vi "Condition.vi"(8 "error in":errorcluster, 11 "Actor in":refnum<class "Actor.lvclass">) -> (0 "error out":errorcluster, 3 "Actor out":refnum<class "Actor.lvclass">)   [LabVIEW 2020, in "_Rescript.lvlib" / "Actor.lvlib" / "Actor.lvclass"]
uses:
  Actor.lvclass
  Actor.lvclass/Actor.ctl
  Condition Delete Controls.vi
  Condition Terminal Attributes.vi
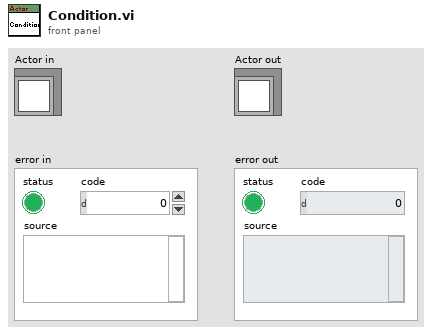
[diagram p1: front panel]
types:
  T1 = typedef "_Rescript.lvlib/Actor.lvlib/Actor.lvclass/Name.ctl" = cluster{"Init Actor VI (Lib)":refnum<vi>}
  T2 = typedef "_Rescript.lvlib/Terminals.ctl" = set{i32}
  T3 = typedef "_Rescript.lvlib/Actor.lvlib/Actor.lvclass/Name Actor.ctl" = cluster{"Init Actor VI (Class)":refnum<vi>, "Init Actor VI (Lib)":refnum<vi>, "Terminal Attributes (Init)":T4}
  T4 = typedef "_Rescript.lvlib/Terminal Attributes.ctl" = map{i32, T5}
  T5 = typedef "_Rescript.lvlib/Attributes.ctl" = cluster{"Control":refnum<vi>, "Wire Rule":enum16{"Invalid Wire Rule", "Required", "Recommended", "Optional", "Dynamic Dispatch"}}
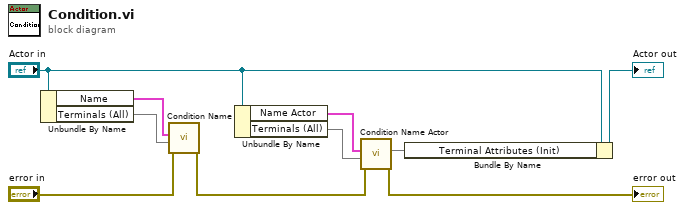
[diagram p0: block diagram]
diagram:
  n1 = Unbundle By Name("Actor in") -> ("Name"=w10:T1, "Terminals (All)"=w9:T2)
  n2 = call "Condition Name.vi"("error in"="error in", "Terminals (All)"=w9, "Name"=w10) -> ("error out"=w7:errorcluster)  [unwired: 8 in]
  n3 = Unbundle By Name("Actor in") -> ("Name Actor"=w2:T3, "Terminals (All)"=w1:T2)
  n4 = call "Condition Name Actor.vi"("error in"=w7, "Terminals (All)"=w1, "Name Actor"=w2) -> ("error out"=→"error out":errorcluster, "Terminal Attributes (Init)"=w4:T4)  [unwired: 7 in]
  n5 = Bundle By Name(cluster="Actor in", "Terminal Attributes (Init)"=w4) -> (→"Actor out":refnum<class "Actor.lvclass">)
